vi "Execute.vi"(6 "commandTimeout":i32=-1, 7 "CommandType":i32(ring)=-1 items=["Text"=1, "StoredProcedure"=4, "TableDirect"=512], 8 "error in (no error)":errorcluster, 9 "DynamicParameters":refnum<class "DynamicParameters.lvclass">, 10 "sql":string, 11 "PGJDPMapper in":refnum<class "Mapper.lvclass">) -> (0 "error out":errorcluster, 2 "affectedRows":i32, 3 "PGJDPMapper out":refnum<class "Mapper.lvclass">)   [LabVIEW 2020, in "ORM_sqlite_jdp.lvlib" / "Mapper.lvclass"]
uses:
  Mapper.lvclass
  C:/Program Files/National Instruments/LabVIEW 2020/vi.lib/Viviota/shared/ORM.lvlibp/SqlMapper/SqlMapper.lvclass
  <vilib>/Viviota/shared/ORM.lvlibp/DynamicParameters/DynamicParameters.lvclass
  dbc/DBC.lvclass
  PGJDPParameter/Parameter.lvclass
  C:/Program Files/National Instruments/LabVIEW 2020/vi.lib/Viviota/shared/ORM.lvlibp/DynamicParameters/DynamicParameters.lvclass
  <vilib>/Viviota/shared/ORM.lvlibp/SqlMapper/Read DbConnection.vi
  dbc/Read Connection.vi
  <vilib>/Viviota/shared/ORM.lvlibp/DynamicParameters/Read ParameterNames.vi
  <vilib>/Viviota/shared/ORM.lvlibp/DynamicParameters/Read ParameterValues.vi
  <vilib>/Viviota/shared/ORM.lvlibp/DbConnection/DbConnection.lvclass
  <vilib>/drjdpowell/SQLite Library/SQL Connection/Connection.lvclass
  Mapper.lvclass/Mapper.ctl
  <vilib>/drjdpowell/SQLite Library/SQL Statement/SQL Statement.lvclass
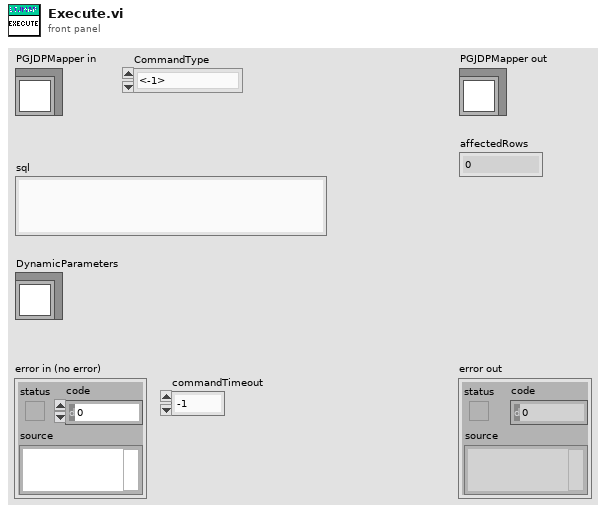
[diagram p1: front panel]
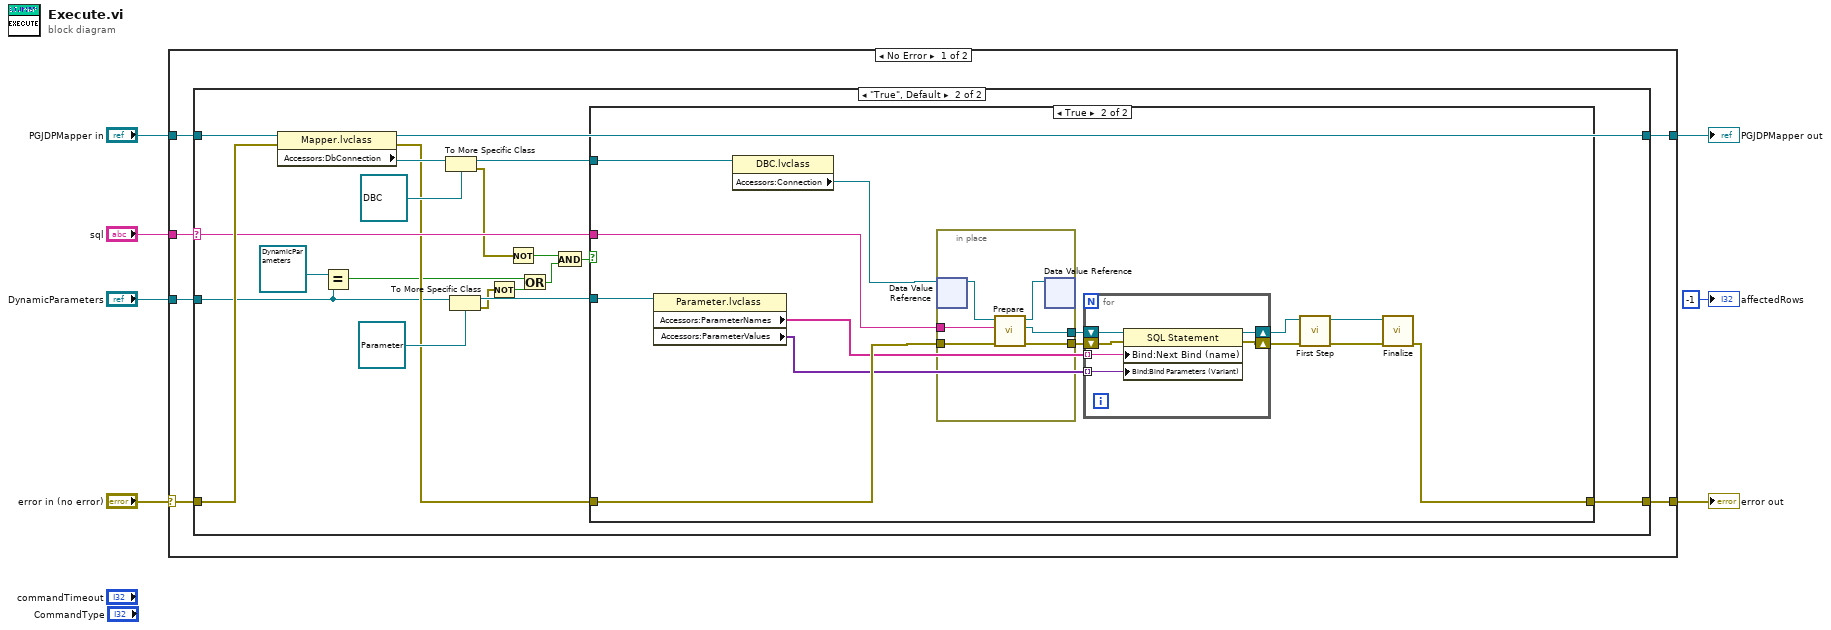
[diagram p0: block diagram]
diagram:
  n1 = case shown="No Error" "error in (no error)" {
    selector: "error in (no error)" -> [w11 w64]
    tunnel: "PGJDPMapper in" -> [w13 w63]
    tunnel: [w12 w63] -> w6
    tunnel: [w10 w64] -> w4
    tunnel: "sql" -> [w9 _]
    tunnel: "DynamicParameters" -> [w8 _]
    frame No Error {
      n2 = case shown="\"True\", Default" w9 {
        selector: w9 -> [_ w28]
        tunnel: w13 -> [w15 w35]
        tunnel: [w15 w34] -> w12
        tunnel: w11 -> [w14 w33]
        tunnel: [w14 w25] -> w10
        tunnel: w8 -> [_ w23]
        frame "" {
        }
        frame "True", Default {
          n3 = property class="Mapper.lvclass"(reference=w35, error in=w33) -> (reference out=w34:refnum<class "Mapper.lvclass">, error out=w26:errorcluster, "Accessors:DbConnection"=w32:refnum<class "DbConnection.lvclass">)
          n4 = Equal?(x=refnum<class "DynamicParameters.lvclass"> refnum ("DynamicParameters"), y=w23) -> (x = y?=w20:bool)
          n5 = To More Specific Class(target class=refnum<class "DBC.lvclass"> refnum ("ORM_pgsql_jdp.lvlib:DBC.lvclass"), reference=w32) -> (specific class reference=w27:refnum<class "DBC.lvclass">, error out=w17:errorcluster)  [unwired: 1 in]
          n6 = To More Specific Class(target class=refnum<class "Parameter.lvclass"> refnum ("ORM_pgsql_jdp.lvlib:PGJDPParameter.lvclass"), reference=w23) -> (specific class reference=w29:refnum<class "Parameter.lvclass">, error out=w21:errorcluster)  [unwired: 1 in]
          n7 = Not(x=w21) -> (.not. x?=w22:bool)
          n8 = Not(x=w17) -> (.not. x?=w16:bool)
          n9 = Or(x=w20, y=w22) -> (x .or. y?=w18:bool)
          n10 = And(x=w16, y=w18) -> (x .and. y?=w19:bool)
          n11 = case shown="True" w19 {
            tunnel: w29 -> [_ w50]
            tunnel: w28 -> [_ w43]
            tunnel: w27 -> [_ w49]
            tunnel: w26 -> [w36 w42]
            tunnel: [w36 w37] -> w25
            frame False {
            }
            frame True {
              n12 = property class="Parameter.lvclass"(reference=w50) -> ("Accessors:ParameterNames"=w41:string[], "Accessors:ParameterValues"=w40:variant[])  [unwired: 1 in, 2 out]
              n13 = property class="DBC.lvclass"(reference=w49) -> ("Accessors:Connection"=w44:refnum<data-value>)  [unwired: 1 in, 2 out]
              n14 = in-place {
                in-place-border: w42 -> [w56]
                in-place-border: w43 -> [w55]
                in-place-border: [w54] -> w48
                in-place-border: [w53] -> w47
                n15 = in-place-dvr #1(w44) -> (w52:refnum<class "Connection.lvclass">)  [unwired: 1 out]
                n16 = call <vilib>:"Prepare.vi"("error in (no error)"=w56, "SQL"=w55, "SQLite Connection in"=w52) -> ("error out"=w54:errorcluster, "SQL Statement"=w53:refnum<class "SQL Statement.lvclass">, "SQLite Connection"=w51:refnum<class "Connection.lvclass">)  [unwired: 4 in, 2 out]
                n17 = in-place-dvr #1(w51) -> ()  [unwired: 2 out]
              }
              n18 = for {
                tunnel: w41 -> [w60] mode=indexing
                tunnel: w40 -> [w59] mode=indexing
                shift-right: [w58] -> w46
                shift-left: w47 -> [w61]
                shift-right: [w57] -> w45
                shift-left: w48 -> [w62]
                n19 = property class="SQL Statement"(reference=w61, error in=w62, "Bind:Next Bind (name)"=w60, "Bind:Bind Parameters (Variant)"=w59) -> (reference out=w58:refnum<class "SQL Statement.lvclass">, error out=w57:errorcluster)
              }
              n20 = call <vilib>:"First Step.vi"("error in (no error)"=w45, "SQL Statement in"=w46) -> ("error out"=w38:errorcluster, "SQL Statement"=w39:refnum<class "SQL Statement.lvclass">)  [unwired: 7 in, 1 out]
              n21 = call <vilib>:"Finalize.vi"("error in (no error)"=w38, "SQL Statement in"=w39) -> ("error out"=w37:errorcluster)  [unwired: 9 in]
            }
          }
        }
      }
    }
    frame Error {
    }
  }
  "error out" <- w4
  "PGJDPMapper out" <- w6
  "affectedRows" <- -1 ("affectedRows")
